vi "pullUpDnControl.Down.vi"(8 "error in (no error)":errorcluster, 11 "RPi Pin":T1) -> (0 "error out":errorcluster, 3 "RPi Pin out":T1)   [LabVIEW 2020, in "wiringPi.lvlib"]
doc: "<b>_______________________________________________________________</b>\n** Author: Juan José Villacorta\n** LabVIEW wrapper for C library <b> wiringPi </b>,\n** https://github.com/WiringPi/WiringPi\n<b>_______________________________________________________________</b>\n\n/*\n * pullUpDownCtrl:\n * Control the internal pull-up/down resistors on a GPIO pin.\n *********************************************************************************\n */"
uses:
  wiringPi.lvlib
  Type Defs/Pull up-down.ctl
  Type Defs/GPIO Pins.ctl
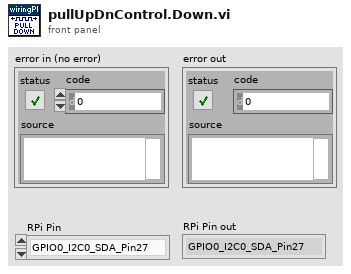
[diagram p1: front panel]
types:
  T1 = typedef "wiringPi.lvlib/GPIO Pins.ctl" = enum32{"GPIO0_I2C0_SDA_Pin27", "GPIO1_I2C0_SDA1_Pin28", "GPIO2_I2C1_SDA_Pin3", "GPIO3_I2C1_SCL_Pin5", "GPIO4_GPCLK0_Pin7", "GPIO5_GPCLK1_Pin29", "GPIO6_GPCLK2_Pin31", "GPIO7_SPI_CE1_N_Pin26", "GPIO8_SPI_CE0_N_Pin24", "GPIO9_SPI0_MISO_Pin21", "GPIO10_SPI0_MOSI_Pin19", "GPIO11_SPI0_CLK_Pin23", "GPIO12_PWM0_Pin32", "GPIO13_PWM1_Pin33", "GPIO14_TXD0_Pin8", "GPIO15_RXD0_Pin10", "GPIO16_Pin36", "GPIO17_Pin11", "GPIO18_PWM0_Pin12", "GPIO19_PWM1_Pin35", "GPIO20_GPCLK0_Pin38", "GPIO21_GPCLK1_Pin40", "GPIO22_Pin15", "GPIO23_Pin16", "GPIO24_Pin18", "GPIO25_Pin22", "GPIO26_Pin37", "GPIO27_Pin13"}
  T2 = typedef "wiringPi.lvlib/Pull up-down.ctl" = enum16{"Off", "Down", "Up"}
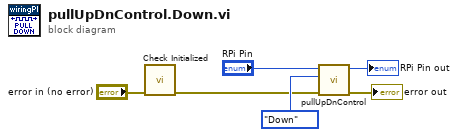
[diagram p0: block diagram]
diagram:
  n1 = call "Check Initialized.vi"("error in (no error)"="error in (no error)") -> ("error out"=w1:errorcluster)  [unwired: 10 in]
  n2 = call "pullUpDnControl.vi"("error in (no error)"=w1, "Up-Down-Off"=Pull_up-down."Down" ("Pull Up-Down Ctrl"), "RPi Pin"="RPi Pin") -> ("error out"=→"error out":errorcluster, "RPi Pin out"=→"RPi Pin out":T1)  [unwired: 7 in]
